vi "GDSIconEditor_FindPrefixInfo.vi"(0 "_VIPath":path, 9 "Folder":path, 11 "error in (no error)":errorcluster) -> (4 "FolderFiles":path[](array[path]), 6 "Prefix":string, 8 "Separator":string, 10 "name":string, 14 "FilePreFix+Separtor":string, 15 "error out":errorcluster)   [LabVIEW 2020]
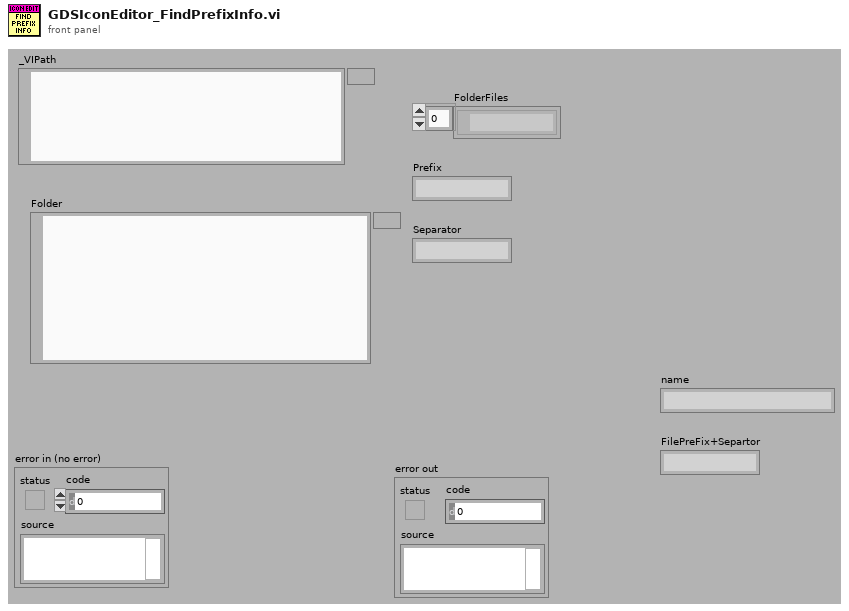
[diagram p1: front panel]
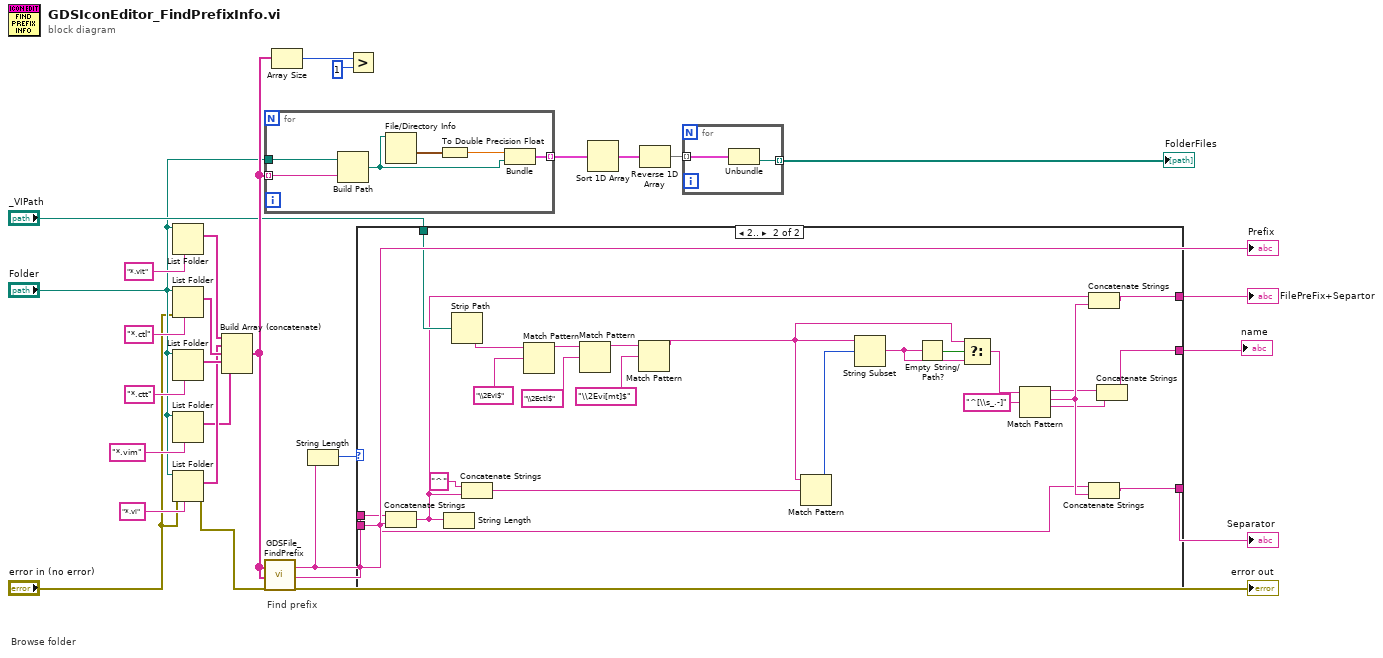
[diagram p0: block diagram]
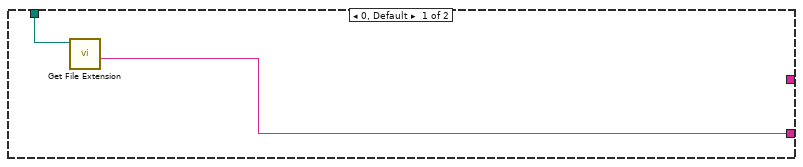
[diagram p2: hidden frame]
diagram:
  # "Browse folder"
  # "Find prefix"
  n1 = List Folder(path="Folder", pattern="*.vit") -> (filenames=w24:string[])  [unwired: 2 in, 3 out]
  n2 = List Folder(path="Folder", pattern="*.ctl", error in="error in (no error)") -> (filenames=w25:string[])  [unwired: 1 in, 3 out]
  n3 = List Folder(path="Folder", pattern="*.ctt") -> (filenames=w26:string[])  [unwired: 2 in, 3 out]
  n4 = List Folder(path="Folder", pattern="*.vim") -> (filenames=w1:string[])  [unwired: 2 in, 3 out]
  n5 = List Folder(path="Folder", pattern="*.vi", error in="error in (no error)") -> (filenames=w16:string[], error out=w15:errorcluster)  [unwired: 1 in, 2 out]
  n6 = Build Array (concatenate)(w24, w16, w25, w26, w1) -> (w20:string[])
  n7 = for {
    tunnel: "Folder" -> [w34]
    tunnel: w20 -> [w33] mode=indexing
    tunnel: [w31] -> w17 mode=indexing
    n8 = Build Path(base path=w34, name or relative path=w33) -> (appended path=w32:path)
    n9 = File/Directory Info(path=w32) -> (last mod=w30:timestamp)  [unwired: 1 in, 6 out]
    n10 = To Double Precision Float(number=w30) -> (double precision float=w29:dbl)
    n11 = Bundle(w29, "appended path"=w32) -> (w31:cluster{dbl, "appended path":path})  [unwired: 1 in]
  }
  n12 = call "GDSFile_FindPrefix.vi"("Filenames as references"=w20, "Filenames to search"=w20, "error in (no error)"=w15) -> ("Prefix"=w6:string, "Separator"=w9:string, "error out"=→"error out":errorcluster)  [unwired: 14 in]
  "Prefix" <- w6
  n13 = Array Size(array=w20) -> (size(s)=w12:i32)
  n14 = String Length(string=w6) -> (length=w5:i32)
  n15 = Greater?(x=w12, y=1) -> ()  [unwired: 1 out]
  n16 = case shown="2.." w5 {
    tunnel: "_VIPath" -> [w36 w60]
    tunnel: [_ w45] -> w10
    tunnel: w9 -> [_ w43]
    tunnel: [_ w42] -> w8
    tunnel: [w35 w38] -> w7
    tunnel: w6 -> [_ w37]
    frame 0, Default {
      n17 = call <vilib>:"Get File Extension.vi"("file"=w36) -> ("filename without extension"=w35:string)  [unwired: 6 in, 4 out]
    }
    frame 2.. {
      n18 = Concatenate Strings(w37, w43) -> (w46:string)
      n19 = String Length(string=w46) -> ()  [unwired: 1 out]
      n20 = Strip Path(path=w60) -> (name=w52:string)  [unwired: 1 out]
      n21 = Concatenate Strings("^", w46) -> (w53:string)
      n22 = Match Pattern(string=w52, regular expression="\\2Evi$") -> (before substring=w57:string)  [unwired: 1 in, 3 out]
      n23 = Match Pattern(string=w57, regular expression="\\2Ectl$") -> (before substring=w56:string)  [unwired: 1 in, 3 out]
      n24 = Match Pattern(string=w56, regular expression="\\2Evi[mt]$") -> (before substring=w50:string)  [unwired: 1 in, 3 out]
      n25 = Match Pattern(string=w50, regular expression=w53) -> (offset past match=w48:i32)  [unwired: 1 in, 3 out]
      n26 = String Subset(string=w50, offset (0)=w48) -> (substring=w49:string)  [unwired: 1 in]
      n27 = Empty String/Path?(string/path=w49) -> (empty?=w51:bool)
      n28 = Select(t=w50, s=w51, f=w49) -> (s? t:f=w39:string)
      n29 = Match Pattern(string=w39, regular expression="^[\\s_.-]") -> (before substring=w41:string, match substring=w44:string, after substring=w40:string)  [unwired: 1 in, 1 out]
      n30 = Concatenate Strings(w46, w44) -> (w45:string)
      n31 = Concatenate Strings(w43, w44) -> (w42:string)
      n32 = Concatenate Strings(w41, w40) -> (w38:string)
    }
  }
  "FilePreFix+Separtor" <- w10
  "name" <- w7
  "Separator" <- w8
  n33 = Sort 1D Array(array=w17) -> (sorted array=w18:cluster{dbl, "appended path":path}[])
  n34 = Reverse 1D Array(array=w18) -> (reversed array=w27:cluster{dbl, "appended path":path}[])
  n35 = for {
    tunnel: w27 -> [w62] mode=indexing
    tunnel: [w61] -> w28 mode=indexing
    n36 = Unbundle(w62) -> ("appended path"=w61:path)  [unwired: 1 out]
  }
  "FolderFiles" <- w28
